vi "Write.vi"(0 "HANDLE":u32, 1 "DATOS":u8[](array[numeric]), 3 "error in (no error)":errorcluster) -> (7 "OUT":i32, 10 "error out":errorcluster)   [LabVIEW 2017, in "HID_ARZ.lvlib"]
doc: "WRITE Write;"
uses:
  HID_ARZ.lvlib
  <userlib>/HID_ARZ/mcHID.dll
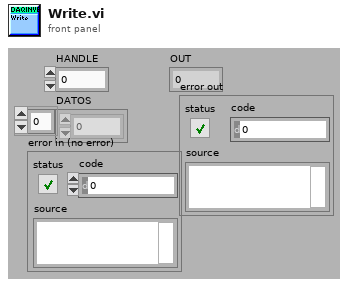
[diagram p1: front panel]
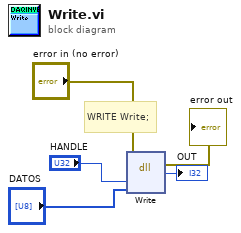
[diagram p0: block diagram]
diagram:
  # "WRITE Write;"
  n1 = dll-call lib="C:/Program Files (x86)/National Instruments/LabVIEW 2017/user.lib/HID_ARZ/mcHID.dll" fn="Write"(error in="error in (no error)", "HANDLE"="HANDLE", "DATOS"="DATOS") -> (error out=→"error out":errorcluster, "OUT"=→"OUT":i32)  [unwired: 4 in, 1 out]
